vi "GetContextHelpInfo.vi"(0 "reference":refnum<class "ClassNode.lvclass">, 1 "MousePos":T1 {"y" format="%.2f"; "x" format="%.2f"}, 5 "error in (no error)":errorcluster) -> (14 "reference out":refnum<class "ClassNode.lvclass">, 15 "ContextHelpInfoExist":bool, 16 "ContextHelpInfo":variant, 19 "error out":errorcluster)   [LabVIEW 2020, in "ClassNode.lvclass"]
doc: "GetContextHelpInfo"
uses:
  <resource>/Framework/Providers/Open_GDS/UML/ClassNode_class/ClassNode.lvclass
  C:/Program Files (x86)/National Instruments/LabVIEW 2020/resource/Framework/Providers/Open_GDS/UML/RectangularNode_class/RectangularNode.lvclass
  <resource>/Framework/Providers/Open_GDS/UML/General/Point/Point Point2D.ctl
  <resource>/Framework/Providers/Open_GDS/UML/MultiLineString_class/MultiLineString.lvclass
  <resource>/Framework/Providers/Open_GDS/ClassProviders/Provider_BaseClassInterface/ClassReader_class/ClassReader.lvclass
  <resource>/Framework/Providers/Open_GDS/UML/RectangularNode_class/RectangularNode.lvclass
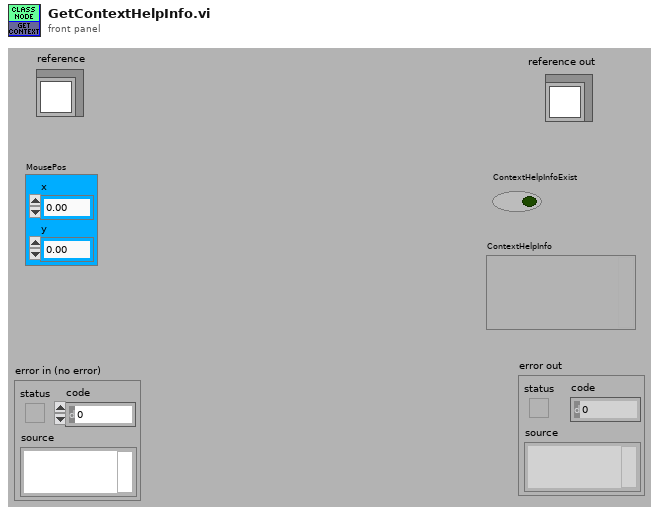
[diagram p1: front panel]
types:
  T1 = typedef "Point Point2D.ctl" = cluster{"x":dbl, "y":dbl}
  T2 = typedef "ClassNode.lvclass/ObjectAttributes.ctl" = cluster{"midHeight":dbl, "botHeight":dbl, "name":refnum<class "MultiLineString.lvclass">, "attributes":refnum<class "MultiLineString.lvclass">, "methods":refnum<class "MultiLineString.lvclass">, "DEFAULT_COMPARTMENT_HEIGHT":i32, "DEFAULT_WIDTH":i32, "DEFAULT_HEIGHT":i32, "showMethods":bool, "showAttributes":bool, "ClassPath":path}
  T3 = typedef "RectangularNode.lvclass/ObjectAttributes.ctl" = cluster{"bounds":T4}
  T4 = typedef "Rectangle Rectangle2D.ctl" = cluster{"x":dbl, "y":dbl, "width":dbl, "height":dbl}
  T5 = typedef "imagedata.ctl" = cluster{"image type":i32, "image depth":i32, "image":u8[], "mask":u8[], "colors":u32[], "Rectangle":cluster{"left":i16, "top":i16, "right":i16, "bottom":i16}}
  T6 = cluster{"text":string, "new picture":picture, "Description":string}
  T7 = cluster{"text":string, "empty picture":picture, "Description":string}
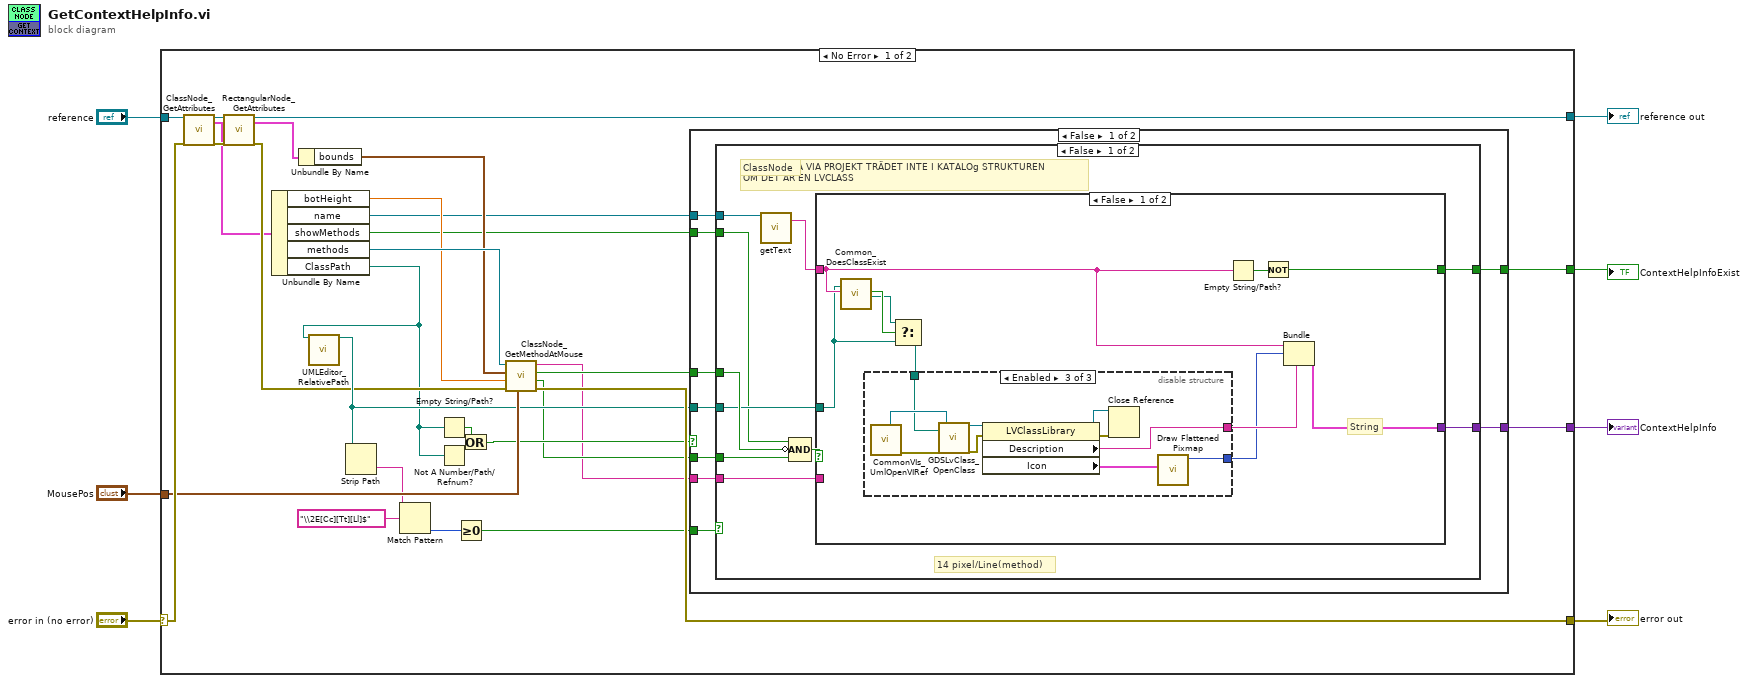
[diagram p0: block diagram]
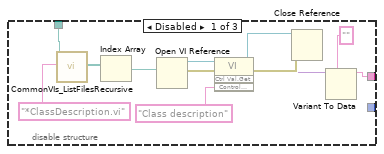
[diagram p2: hidden frame]
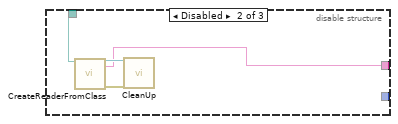
[diagram p3: hidden frame]
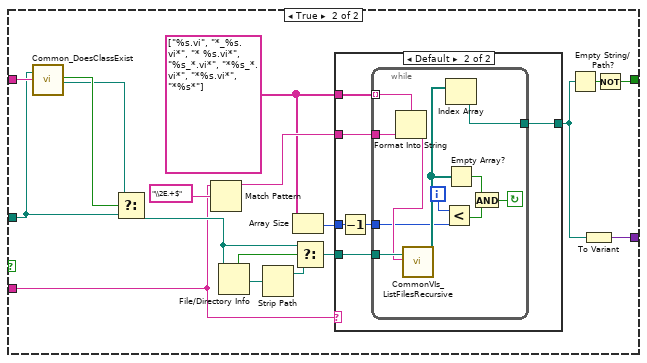
[diagram p4: hidden frame]
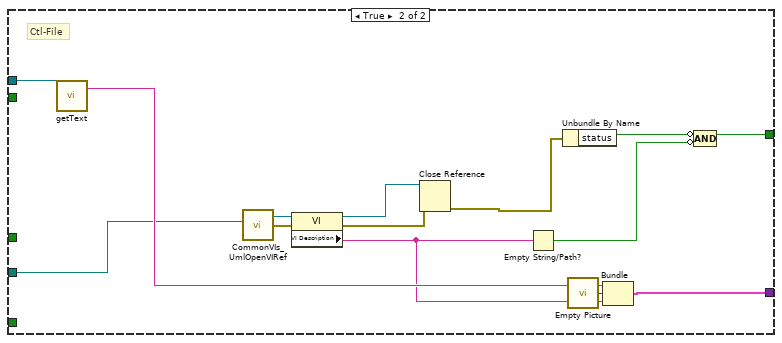
[diagram p6: hidden frame]
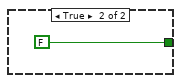
[diagram p7: hidden frame]
diagram:
  n1 = case shown="No Error" "error in (no error)" {
    selector: "error in (no error)" -> [w36 w142]
    tunnel: "reference" -> [w35 w143]
    tunnel: [w32 w142] -> w5
    tunnel: [w11 w143] -> w4
    tunnel: "MousePos" -> [w33 _]
    tunnel: [w31 _] -> w2
    tunnel: [w30 _] -> w1
    frame No Error {
      n2 = call <resource>:"ClassNode_GetAttributes.vi"("reference in"=w35, "error in (no error)"=w36) -> ("reference out"=w14:refnum<class "ClassNode.lvclass">, "Data"=w9:T2, "error out"=w13:errorcluster)  [unwired: 1 in, 14 out]
      n3 = call <resource>:"RectangularNode_GetAttributes.vi"("reference in"=w14, "error in (no error)"=w13) -> ("reference out"=w11:refnum<class "ClassNode.lvclass">, "Data"=w10:T3, "error out"=w12:errorcluster)  [unwired: 14 in, 1 out]
      n4 = Unbundle By Name(w9) -> ("botHeight"=w28:dbl, "name"=w25:refnum<class "MultiLineString.lvclass">, "showMethods"=w26:bool, "methods"=w34:refnum<class "MultiLineString.lvclass">, "ClassPath"=w8:path)
      n5 = Unbundle By Name(w10) -> ("bounds"=w29:T4)
      n6 = call <resource>:"UMLEditor_RelativePath.vi"("Path In"=w8) -> ("ConvertToAbsolutePath(If possible)"=w17:path)  [unwired: 1 in, 17 out]
      n7 = Strip Path(path=w17) -> (name=w21:string)  [unwired: 1 out]
      n8 = Match Pattern(string=w21, regular expression="\\2E[Cc][Tt][Ll]$") -> (offset past match=w19:i32)  [unwired: 4 out]
      n9 = Empty String/Path?(string/path=w8) -> (empty?=w24:bool)
      n10 = Not A Number/Path/Refnum?(number/path/refnum=w8) -> (NaN/Path/Refnum?=w23:bool)
      n11 = Greater Or Equal To 0?(x=w19) -> (x >= 0?=w18:bool)
      n12 = Or(x=w24, y=w23) -> (x .or. y?=w22:bool)
      n13 = call <resource>:"ClassNode_GetMethodAtMouse.vi"("MousePos"=w33, "error in"=w12, "botHeight"=w28, "bounds"=w29, "methods"=w34) -> ("error out"=w32:errorcluster, "MethodSelected"=w16:bool, "NoMmethodsExists"=w27:bool, "MEthodName"=w15:string)  [unwired: 1 in]
      n14 = case shown="False" w22 {
        tunnel: [w45 _] -> w31
        tunnel: [w44 FALSE] -> w30
        tunnel: w27 -> [w43 _]
        tunnel: w26 -> [w41 _]
        tunnel: w25 -> [w40 _]
        tunnel: w17 -> [w42 _]
        tunnel: w18 -> [w39 _]
        tunnel: w16 -> [w38 _]
        tunnel: w15 -> [w37 _]
        frame False {
          n15 = case shown="False" w39 {
            tunnel: [w55 w133] -> w45
            tunnel: [w54 w135] -> w44
            tunnel: w43 -> [w52 _]
            tunnel: w42 -> [w51 w129]
            tunnel: w41 -> [w46 _]
            tunnel: w40 -> [w50 w132]
            tunnel: w38 -> [w48 _]
            tunnel: w37 -> [w47 _]
            frame False {
              # "MÅSTE SÖKA VIA PROJEKT TRÄDET INTE I KATALOg STRUKTUREN\nOM DET ÄR EN LVCLASS"
              # "ClassNode"
              # "14 pixel/Line(method)"
              n16 = call-dynamic "getText.vi"("reference"=w50) -> ("text"=w49:string)  [unwired: 1 in, 17 out]
              n17 = Compound Arithmetic op=AND(w46, invert w52, w48) -> (w53:bool)
              n18 = case shown="False" w53 {
                tunnel: w51 -> [w58 w106]
                tunnel: [w64 w108] -> w55
                tunnel: [w62 w101] -> w54
                tunnel: w49 -> [w59 w107]
                tunnel: w47 -> [_ w92]
                frame False {
                  # "String"
                  n19 = call <resource>:"Common_DoesClassExist.vi"("ClassPath"=w58, "ClassName"=w59) -> ("llb-class"=w61:bool, "llb/LvCLass-Path"=w60:path)  [unwired: 16 out]
                  n20 = Select(t=w60, s=w61, f=w58) -> (s? t:f=w57:path)
                  n21 = disable-structure shown="Enabled" {
                    disable-tunnel: [w67 w78 w87] -> w65
                    disable-tunnel: w57 -> [w66 w79 w89]
                    disable-tunnel: [_ _ w82] -> w56
                    frame Disabled {
                      n22 = call <resource>:"CommonVIs_ListFilesRecursive.vi"("directory path"=w66, "FileSearchPattern"="*ClassDescription.vi") -> ("Files"=w77:path[])  [unwired: 14 in, 3 out]
                      n23 = Index Array(array=w77) -> (element=w75:path)  [unwired: 1 in]
                      n24 = Open VI Reference(vi path=w75) -> (vi reference=w73:refnum<vi>, error out=w74:errorcluster)  [unwired: 5 in]
                      n25 = invoke class="VI" method="Ctrl Val.Get"(reference=w73, error in=w74, "Control Name"="Class description") -> (reference out=w71:refnum<vi>, error out=w70:errorcluster, "Get Control Value Variant"=w69:variant)  [unwired: 1 in, 1 out]
                      n26 = Close Reference(reference=w71, error in (no error)=w70) -> ()  [unwired: 1 out]
                      n27 = Variant To Data(type="", Variant=w69) -> (data=w67:string)  [unwired: 1 in, 1 out]
                    }
                    frame Disabled {
                      n28 = call <resource>:"CreateReaderFromClass.vi"("ClassPath/LvClassRef"=w79) -> ("ClassReader"=w80:refnum<class "ClassReader.lvclass">, "Description"=w78:string, "error out"=w81:errorcluster)  [unwired: 1 in, 15 out]
                      n29 = call-dynamic "CleanUp.vi"("reference in"=w80, "error in (no error)"=w81) -> ()  [unwired: 18 out]
                    }
                    frame Enabled {
                      n30 = call <resource>:"CommonVIs_UmlOpenVIRef.vi"() -> ("error out"=w91:errorcluster, "AppRefOut"=w90:refnum<vi>)  [unwired: 8 in, 2 out]
                      n31 = call <resource>:"GDSLvClass_OpenClass.vi"("ClassToOpen"=w89, "error in (no error)"=w91, "Project/ApplicationRef(If empty, currect active project will be used)"=w90) -> ("LVClass.Open"=w88:refnum<vi>, "error out"=w86:errorcluster)  [unwired: 15 in]
                      n32 = property class="LVClassLibrary"(reference=w88, error in=w86) -> (reference out=w85:refnum<vi>, error out=w84:errorcluster, "Description"=w87:string, "Icon"=w83:T5)
                      n33 = Close Reference(reference=w85, error in (no error)=w84) -> ()  [unwired: 1 out]
                      n34 = call <vilib>:"Draw Flattened Pixmap.vi"("image data"=w83) -> ("new picture"=w82:picture)  [unwired: 8 in]
                    }
                  }
                  n35 = Empty String/Path?(string/path=w59) -> (empty?=w63:bool)
                  n36 = Not(x=w63) -> (.not. x?=w62:bool)
                  n37 = Bundle("text"=w59, "new picture"=w56, "Description"=w65) -> (w64:T6)  [unwired: 1 out]
                }
                frame True {
                  w97 = string[] ["%s.vi", "*_%s.vi*", "* %s.vi*", "%s_*.vi*", "*%s_*.vi*", "*%s.vi*", "*%s*"]
                  n38 = call <resource>:"Common_DoesClassExist.vi"("ClassPath"=w106, "ClassName"=w107) -> ("llb-class"=w105:bool, "llb/LvCLass-Path"=w104:path)  [unwired: 16 out]
                  n39 = Select(t=w104, s=w105, f=w106) -> (s? t:f=w93:path)
                  n40 = Match Pattern(string=w92, regular expression="\\2E.+$") -> (before substring=w98:string)  [unwired: 4 out]
                  n41 = File/Directory Info(path=w93) -> (path out=w95:path, directory=w100:bool)  [unwired: 1 in, 5 out]
                  n42 = Strip Path(path=w95) -> (stripped path=w94:path)  [unwired: 1 out]
                  n43 = Array Size(array=w97) -> (size(s)=w96:i32)
                  n44 = Select(t=w93, s=w100, f=w94) -> (s? t:f=w99:path)
                  n45 = case shown="Default" w92 {
                    tunnel: [_ w112] -> w103
                    tunnel: w99 -> [_ w115]
                    tunnel: w97 -> [_ w114]
                    tunnel: w98 -> [_ w113]
                    tunnel: w96 -> [_ w111]
                    frame "" {
                    }
                    frame Default {
                      n46 = Decrement(x=w111) -> (x-1=w110:i32)
                      n47 = while {
                        tunnel: w115 -> [w126]
                        tunnel: w114 -> [w125] mode=indexing
                        tunnel: w113 -> [w124]
                        tunnel: [w123] -> w112
                        tunnel: w110 -> [w119]
                        i -> [w120]
                        stop <- w116 continue-if-true
                        n48 = Format Into String(format string=w125, w124) -> (resulting string=w121:string)  [unwired: 2 in, 1 out]
                        n49 = call <resource>:"CommonVIs_ListFilesRecursive.vi"("directory path"=w126, "FileSearchPattern"=w121) -> ("Files"=w122:path[])  [unwired: 4 in, 13 out]
                        n50 = Less?(x=w120, y=w119) -> (x < y?=w117:bool)
                        n51 = Index Array(array=w122) -> (element=w123:path)  [unwired: 1 in]
                        n52 = Empty Array?(array=w122) -> (empty?=w118:bool)
                        n53 = And(x=w118, y=w117) -> (x .and. y?=w116:bool)
                      }
                    }
                  }
                  n54 = Empty String/Path?(string/path=w103) -> (empty?=w102:bool)
                  n55 = To Variant(anything=w103) -> (Variant=w108:variant)
                  n56 = Not(x=w102) -> (.not. x?=w101:bool)
                }
              }
            }
            frame True {
              # "Ctl-File"
              n57 = call-dynamic "getText.vi"("reference"=w132) -> ("text"=w131:string)  [unwired: 1 in, 17 out]
              n58 = call <resource>:"CommonVIs_UmlOpenVIRef.vi"("ViPath/ViName"=w129) -> ("error out"=w128:errorcluster, "vi reference"=w127:refnum<vi>)  [unwired: 7 in, 2 out]
              n59 = property class="VI"(reference=w127, error in=w128) -> (reference out=w140:refnum<vi>, error out=w139:errorcluster, "VI Description"=w130:string)
              n60 = Close Reference(reference=w140, error in (no error)=w139) -> (error out=w138:errorcluster)
              n61 = Empty String/Path?(string/path=w130) -> (empty?=w136:bool)
              n62 = Unbundle By Name(w138) -> ("status"=w137:bool)
              n63 = call "Empty Picture"() -> ("empty picture"=w134:picture)
              n64 = Bundle("text"=w131, "empty picture"=w134, "Description"=w130) -> (w133:T7)  [unwired: 1 out]
              n65 = Compound Arithmetic op=AND(invert w137, invert w136) -> (w135:bool)
            }
          }
        }
        frame True {
        }
      }
    }
    frame Error {
    }
  }
  "reference out" <- w4
  "error out" <- w5
  "ContextHelpInfo" <- w2
  "ContextHelpInfoExist" <- w1
